vi "Cleanup.vi"(8 "error in (no error)":errorcluster, 11 "NodeRef In":refnum<data-value>) -> (0 "error out":errorcluster)   [LabVIEW 2020, in "PicoG-ParserLexer.lvlib" / "Node.lvclass"]
uses:
  Node.lvclass
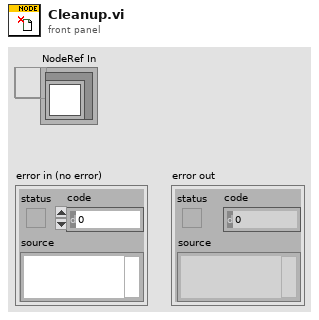
[diagram p1: front panel]
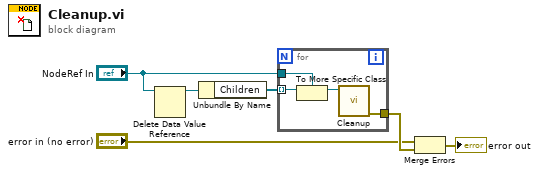
[diagram p0: block diagram]
diagram:
  n1 = Delete Data Value Reference(data value reference="NodeRef In") -> (data value=w5:refnum<class "Node.lvclass">)  [unwired: 1 in, 1 out]
  n2 = Unbundle By Name(w5) -> ("Children"=w1:refnum<data-value>[])
  n3 = for {
    tunnel: [w10] -> w6
    tunnel: "NodeRef In" -> [w8]
    tunnel: w1 -> [w7] mode=indexing
    n4 = To More Specific Class(target class=w8, reference=w7) -> (specific class reference=w9:refnum<data-value>)  [unwired: 1 in, 1 out]
    n5 = call "Cleanup.vi"("NodeRef In"=w9) -> ("error out"=w10:errorcluster)  [unwired: 10 in]
  }
  n6 = Merge Errors("error in (no error)", w6) -> (→"error out":errorcluster)
